vi "addEdge.vi"(0 "reference":refnum<class "CallNode.lvclass">, 1 "egde":refnum<class "AbstractEdge.lvclass">, 2 "p1":T1 {"y" format="%.2f"; "x" format="%.2f"}, 3 "p2":T1 {"y" format="%.2f"; "x" format="%.2f"}, 5 "error in (no error)":errorcluster) -> (14 "reference out":refnum<class "CallNode.lvclass">, 15 "edgeHasEndNode":bool, 19 "error out":errorcluster)   [LabVIEW 2020, in "CallNode.lvclass"]
uses:
  <resource>/Framework/Providers/Open_GDS/UML/CallNode_class/CallNode.lvclass
  C:/Program Files (x86)/National Instruments/LabVIEW 2020/resource/Framework/Providers/Open_GDS/UML/AbstractNode_class/AbstractNode.lvclass
  C:/Program Files (x86)/National Instruments/LabVIEW 2020/resource/Framework/Providers/Open_GDS/UML/RectangularNode_class/RectangularNode.lvclass
  <resource>/Framework/Providers/Open_GDS/UML/AbstractEdge_class/AbstractEdge.lvclass
  <resource>/Framework/Providers/Open_GDS/UML/General/Point/Point Point2D.ctl
  <resource>/Framework/Providers/Open_GDS/UML/ImplicitParameterNode_class/ImplicitParameterNode.lvclass
  <resource>/Framework/Providers/Open_GDS/UML/SegmentedLineEdge_class/SegmentedLineEdge.lvclass
  <resource>/Framework/Providers/Open_GDS/UML/RectangularNode_class/RectangularNode.lvclass
  <resource>/Framework/Providers/Open_GDS/UML/AbstractNode_class/AbstractNode.lvclass
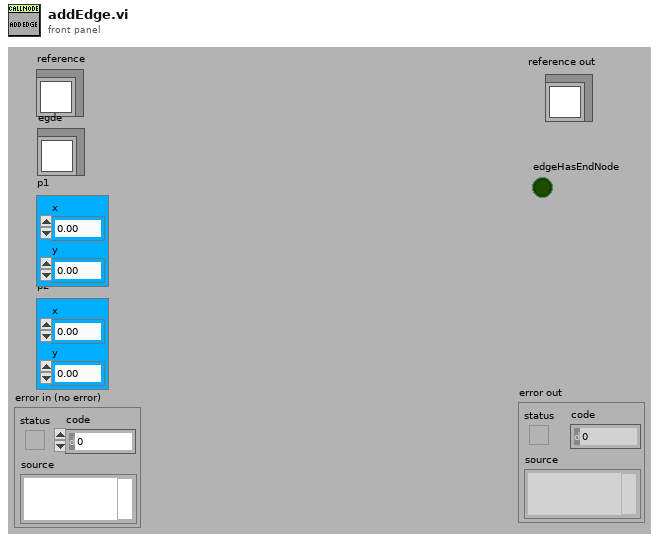
[diagram p1: front panel]
types:
  T1 = typedef "Point Point2D.ctl" = cluster{"x":dbl, "y":dbl}
  T2 = typedef "AbstractNode.lvclass/ObjectAttributes.ctl" = cluster{"parent":refnum<class "AbstractNode.lvclass">, "children":refnum<class "AbstractNode.lvclass">[], "Hidden":bool}
  T3 = typedef "Rectangle Rectangle2D.ctl" = cluster{"x":dbl, "y":dbl, "width":dbl, "height":dbl}
  T4 = typedef "CallNode.lvclass/ObjectAttributes.ctl" = cluster{"objectCallNodeRef":refnum<class "AbstractNode.lvclass">, "signaled":bool, "openBottom":bool, "DEFAULT_WIDTH":i32, "DEFAULT_HEIGHT":i32, "CALL_YGAP":i32}
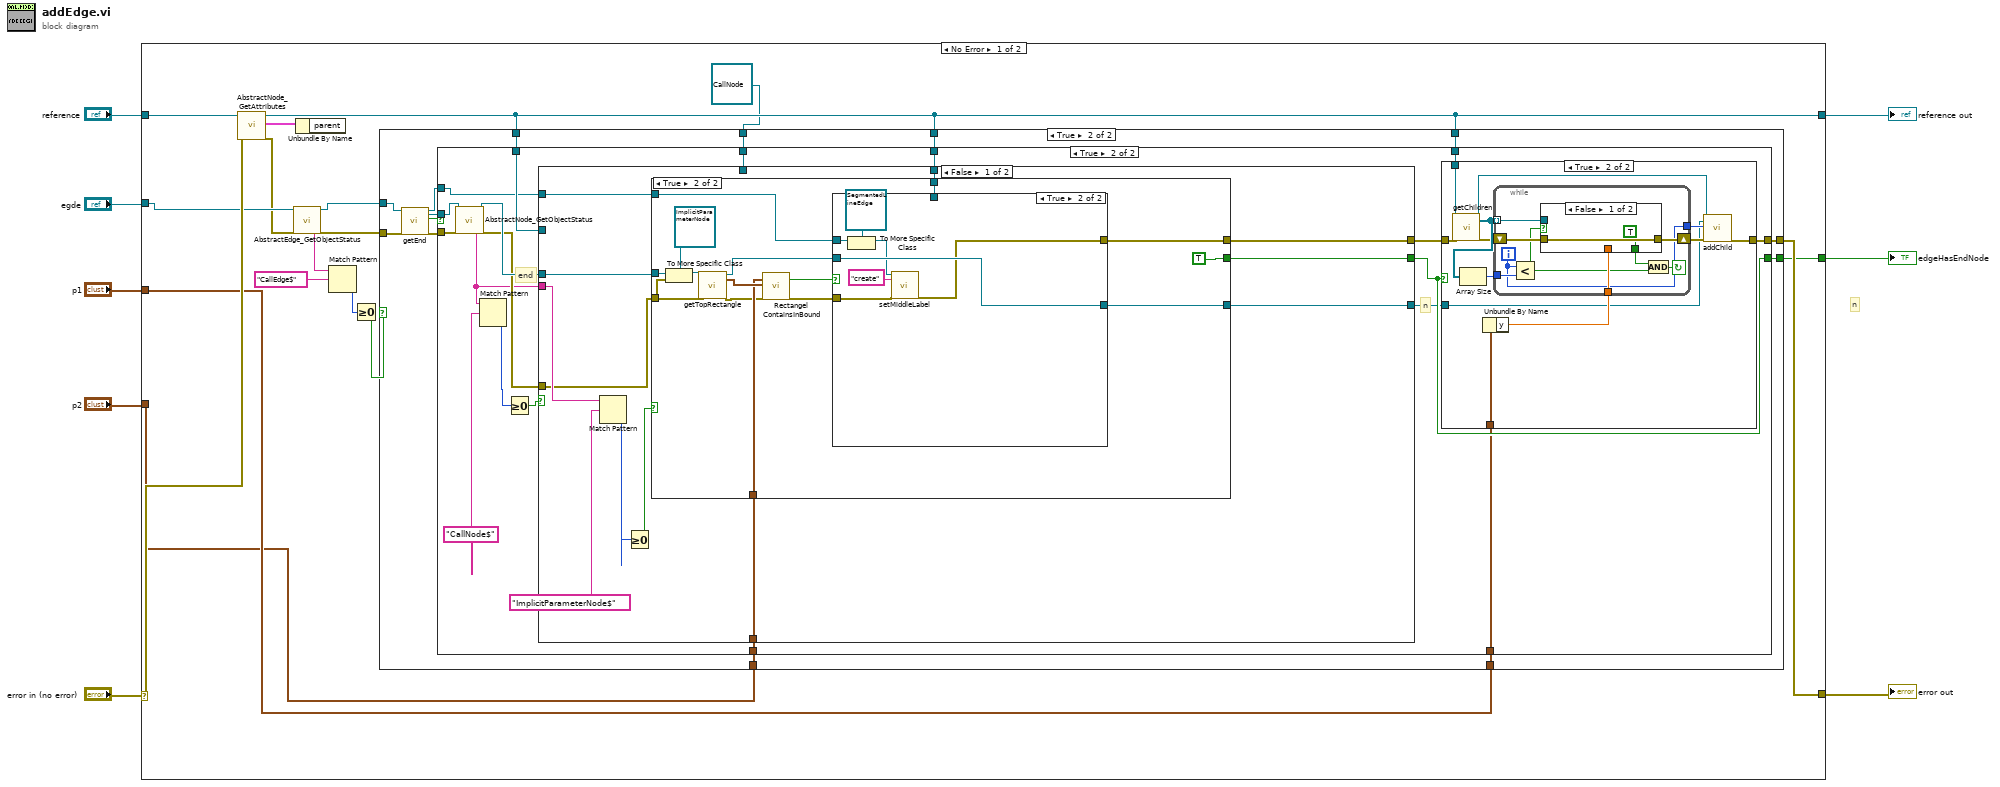
[diagram p0: block diagram]
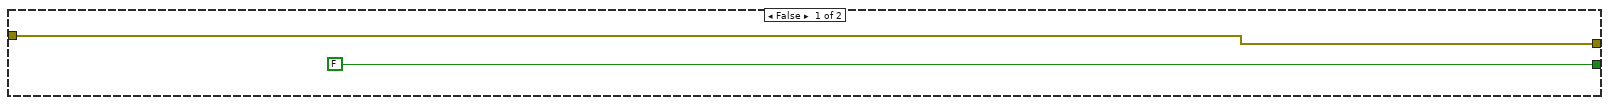
[diagram p2: hidden frame]
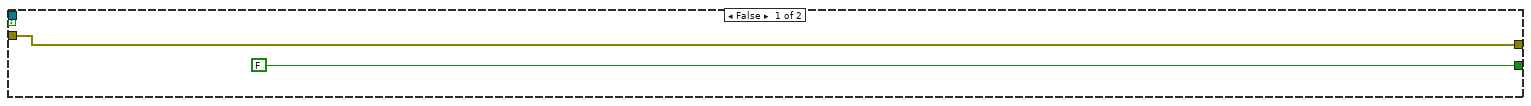
[diagram p3: hidden frame]
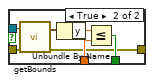
[diagram p5: hidden frame]
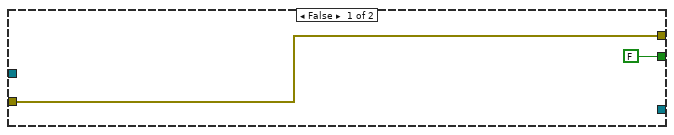
[diagram p6: hidden frame]
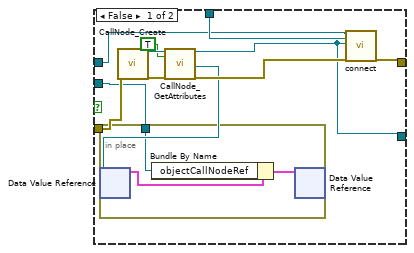
[diagram p7: hidden frame]
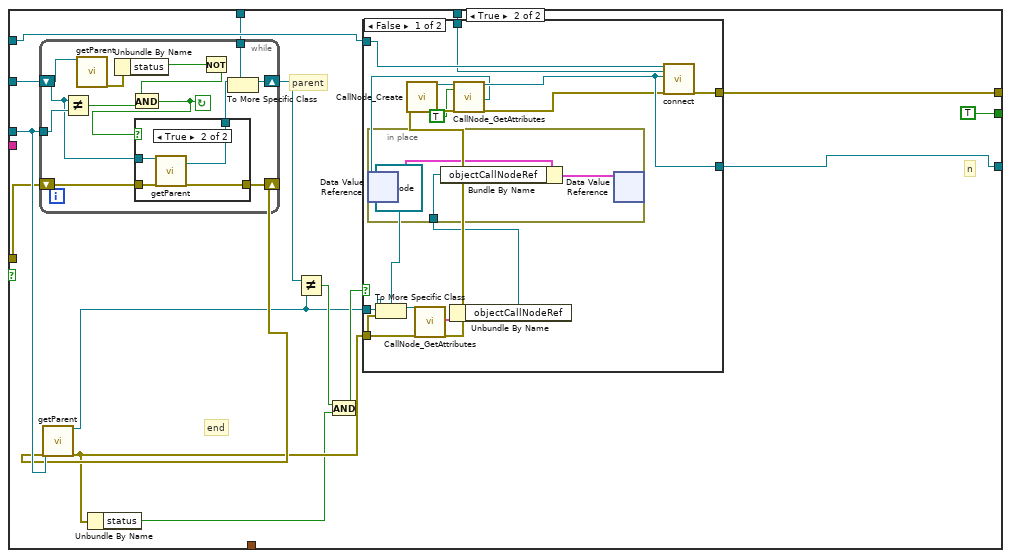
[diagram p8: hidden frame]
diagram:
  # "n"
  n1 = case shown="No Error" "error in (no error)" {
    selector: "error in (no error)" -> [w22 w199]
    tunnel: "reference" -> [w25 w200]
    tunnel: [w24 w199] -> w7
    tunnel: [w23 w200] -> w6
    tunnel: "egde" -> [w21 _]
    tunnel: [w20 _] -> w3
    tunnel: "p1" -> [w19 _]
    tunnel: "p2" -> [w18 _]
    frame No Error {
      n2 = call <resource>:"AbstractNode_GetAttributes.vi"("reference in"=w25, "error in (no error)"=w22) -> ("reference out"=w23:refnum<class "CallNode.lvclass">, "Data"=w10:T2, "error out"=w14:errorcluster)  [unwired: 14 in, 1 out]
      n3 = call <resource>:"AbstractEdge_GetObjectStatus.vi"("reference in"=w21, "error in (no error)"=w14) -> ("Class name"=w9:string, "reference out"=w13:refnum<class "AbstractEdge.lvclass">, "error out"=w12:errorcluster)  [unwired: 15 out]
      n4 = Unbundle By Name(w10) -> ()  [unwired: 1 out]
      n5 = Match Pattern(string=w9, regular expression="CallEdge$") -> (offset past match=w16:i32)  [unwired: 4 out]
      n6 = Greater Or Equal To 0?(x=w16) -> (x >= 0?=w15:bool)
      n7 = case shown="True" w15 {
        tunnel: [FALSE w41] -> w20
        tunnel: w13 -> [_ w40]
        tunnel: w12 -> [w26 w39]
        tunnel: w23 -> [_ w35]
        tunnel: w23 -> [_ w33]
        tunnel: w18 -> [_ w32]
        tunnel: w23 -> [_ w31]
        tunnel: w19 -> [_ w30]
        tunnel: [w26 w29] -> w24
        tunnel: refnum<class "CallNode.lvclass"> refnum ("reference out") -> [_ w28]
        frame False {
        }
        frame True {
          n8 = call-dynamic "getEnd.vi"("reference"=w40, "error in (no error)"=w39) -> ("reference out"=w34:refnum<class "AbstractEdge.lvclass">, "endNode"=w37:refnum<class "AbstractNode.lvclass">, "validNode"=w38:bool, "error out"=w36:errorcluster)  [unwired: 14 in]
          n9 = case shown="True" w38 {
            tunnel: [FALSE w50] -> w41
            tunnel: w37 -> [_ w62]
            tunnel: w36 -> [w42 w61]
            tunnel: w35 -> [_ w57]
            tunnel: w34 -> [_ w54]
            tunnel: w33 -> [_ w53]
            tunnel: w32 -> [_ w51]
            tunnel: w31 -> [_ w49]
            tunnel: w30 -> [_ w47]
            tunnel: [w42 w45] -> w29
            tunnel: w28 -> [_ w44]
            frame False {
            }
            frame True {
              # "n"
              # "end"
              n10 = call <resource>:"AbstractNode_GetObjectStatus.vi"("reference in"=w62, "error in (no error)"=w61) -> ("Class name"=w52:string, "reference out"=w56:refnum<class "AbstractNode.lvclass">, "error out"=w55:errorcluster)  [unwired: 15 out]
              n11 = Match Pattern(string=w52, regular expression="CallNode$") -> (offset past match=w60:i32)  [unwired: 4 out]
              n12 = Greater Or Equal To 0?(x=w60) -> (x >= 0?=w58:bool)
              n13 = case shown="False" w58 {
                tunnel: w57 -> [_ w159]
                tunnel: w56 -> [w100 w158]
                tunnel: w55 -> [w99 w155]
                tunnel: w54 -> [w96 w152]
                tunnel: w53 -> [w95 w151]
                tunnel: w52 -> [w103 _]
                tunnel: [w102 TRUE] -> w50
                tunnel: w51 -> [w98 _]
                tunnel: [w97 w149] -> w46
                tunnel: [w94 w147] -> w48
                tunnel: w44 -> [_ w146]
                frame False {
                  n14 = Match Pattern(string=w103, regular expression="ImplicitParameterNode$") -> (offset past match=w104:i32)  [unwired: 4 out]
                  n15 = Greater Or Equal To 0?(x=w104) -> (x >= 0?=w101:bool)
                  n16 = case shown="True" w101 {
                    tunnel: [FALSE TRUE] -> w102
                    tunnel: w100 -> [_ w110]
                    tunnel: w99 -> [w106 w111]
                    tunnel: w98 -> [_ w120]
                    tunnel: [_ w117] -> w97
                    tunnel: w96 -> [_ w115]
                    tunnel: w95 -> [_ w113]
                    tunnel: [w106 w112] -> w94
                    frame False {
                    }
                    frame True {
                      n17 = To More Specific Class(target class=refnum<class "ImplicitParameterNode.lvclass"> refnum ("reference"), reference=w110, error in=w111) -> (specific class reference=w108:refnum<class "ImplicitParameterNode.lvclass">)  [unwired: 1 out]
                      n18 = call-dynamic "getTopRectangle.vi"("reference"=w108, "error in (no error)"=w111) -> ("reference out"=w116:refnum<class "ImplicitParameterNode.lvclass">, "bounds"=w121:T3, "error out"=w119:errorcluster)  [unwired: 15 in]
                      n19 = call <resource>:"Rectangel ContainsInBound.vi"("point2D"=w120, "bounds"=w121, "error in (no error)"=w119) -> ("contains"=w118:bool, "error out"=w114:errorcluster)  [unwired: 1 in, 14 out]
                      n20 = case shown="True" w118 {
                        tunnel: [w127 w141] -> w117
                        tunnel: w116 -> [w123 w141]
                        tunnel: w115 -> [w128 w138]
                        tunnel: w114 -> [w131 w143]
                        tunnel: w113 -> [w129 _]
                        tunnel: [w126 w140] -> w112
                        frame False {
                          n21 = call <resource>:"CallNode_Create.vi"("error in (no error)"=w131) -> ("reference out"=w133:refnum<class "CallNode.lvclass">, "error out"=w132:errorcluster)  [unwired: 1 in, 16 out]
                          n22 = call <resource>:"CallNode_GetAttributes.vi"("reference in"=w133, "OnlyGetDvrReference(False)"=TRUE, "error in (no error)"=w132) -> ("reference out"=w127:refnum<class "CallNode.lvclass">, "DataRef"=w124:refnum<data-value>, "error out"=w130:errorcluster)  [unwired: 13 in, 1 out]
                          n23 = in-place {
                            in-place-border: w123 -> [w135]
                            n24 = in-place-dvr #1(w124) -> (w136:T4)  [unwired: 1 out]
                            n25 = Bundle By Name(cluster=w136, "objectCallNodeRef"=w135) -> (w134:T4)
                            n26 = in-place-dvr #1(w134) -> ()  [unwired: 2 out]
                          }
                          n27 = call-dynamic "connect.vi"("reference"=w128, "startNode"=w129, "endNode"=w127, "error in (no error)"=w130) -> ("error out"=w126:errorcluster)  [unwired: 14 in, 1 out]
                        }
                        frame True {
                          n28 = To More Specific Class(target class=refnum<class "SegmentedLineEdge.lvclass"> refnum ("reference"), reference=w138) -> (specific class reference=w137:refnum<class "SegmentedLineEdge.lvclass">)  [unwired: 1 in, 1 out]
                          n29 = call-dynamic "setMiddleLabel.vi"("reference"=w137, "middleLabel"="create", "error in (no error)"=w143) -> ("error out"=w140:errorcluster)  [unwired: 15 in, 1 out]
                        }
                      }
                    }
                  }
                }
                frame True {
                  # "parent"
                  # "end"
                  # "n"
                  n30 = while {
                    shift-right: [w185] -> w157
                    shift-left: w159 -> [w184]
                    tunnel: w158 -> [w192]
                    shift-right: [w188] -> w156
                    shift-left: w155 -> [w189]
                    tunnel: w146 -> [w186]
                    stop <- w190 continue-if-true
                    n31 = Not Equal?(x=w184, y=w192) -> (x != y?=w191:bool)
                    n32 = call-dynamic "getParent.vi"("reference"=w184) -> ("error out"=w183:errorcluster)  [unwired: 14 in, 4 out]
                    n33 = Unbundle By Name(w183) -> ("status"=w182:bool)
                    n34 = Not(x=w182) -> (.not. x?=w181:bool)
                    n35 = And(x=w181, y=w191) -> (x .and. y?=w190:bool)
                    n36 = case shown="True" w190 {
                      tunnel: w184 -> [w194 w198]
                      tunnel: [w194 w197] -> w187
                      tunnel: w189 -> [w193 w196]
                      tunnel: [w193 w195] -> w188
                      frame False {
                      }
                      frame True {
                        n37 = call-dynamic "getParent.vi"("reference"=w198, "error in (no error)"=w196) -> ("parentNode"=w197:refnum<class "AbstractNode.lvclass">, "error out"=w195:errorcluster)  [unwired: 13 in, 3 out]
                      }
                    }
                    n38 = To More Specific Class(target class=w186, reference=w187) -> (specific class reference=w185:refnum<class "CallNode.lvclass">)  [unwired: 1 in, 1 out]
                  }
                  n39 = call-dynamic "getParent.vi"("reference"=w158, "error in (no error)"=w156) -> ("reference out"=w150:refnum<class "AbstractNode.lvclass">, "error out"=w145:errorcluster)  [unwired: 13 in, 3 out]
                  n40 = Unbundle By Name(w145) -> ("status"=w144:bool)
                  n41 = Not Equal?(x=w157, y=w150) -> (x != y?=w154:bool)
                  n42 = And(x=w154, y=w144) -> (x .and. y?=w153:bool)
                  n43 = case shown="False" w153 {
                    tunnel: w150 -> [w166 w180]
                    tunnel: [w171 w180] -> w149
                    tunnel: w152 -> [w173 _]
                    tunnel: w151 -> [w172 _]
                    tunnel: w145 -> [w167 w179]
                    tunnel: [w168 w179] -> w147
                    frame False {
                      n44 = To More Specific Class(target class=refnum<class "CallNode.lvclass"> refnum ("reference out"), reference=w166, error in=w167) -> (specific class reference=w165:refnum<class "CallNode.lvclass">)  [unwired: 1 out]
                      n45 = call <resource>:"CallNode_GetAttributes.vi"("reference in"=w165, "error in (no error)"=w167) -> ("Data"=w162:T4, "error out"=w170:errorcluster)  [unwired: 1 in, 15 out]
                      n46 = call <resource>:"CallNode_Create.vi"("error in (no error)"=w170) -> ("reference out"=w175:refnum<class "CallNode.lvclass">, "error out"=w174:errorcluster)  [unwired: 1 in, 16 out]
                      n47 = Unbundle By Name(w162) -> ("objectCallNodeRef"=w160:refnum<class "AbstractNode.lvclass">)
                      n48 = call <resource>:"CallNode_GetAttributes.vi"("reference in"=w175, "OnlyGetDvrReference(False)"=TRUE, "error in (no error)"=w174) -> ("reference out"=w171:refnum<class "CallNode.lvclass">, "DataRef"=w161:refnum<data-value>, "error out"=w169:errorcluster)  [unwired: 13 in, 1 out]
                      n49 = in-place {
                        in-place-border: w160 -> [w177]
                        n50 = in-place-dvr #2(w161) -> (w178:T4)  [unwired: 1 out]
                        n51 = Bundle By Name(cluster=w178, "objectCallNodeRef"=w177) -> (w176:T4)
                        n52 = in-place-dvr #2(w176) -> ()  [unwired: 2 out]
                      }
                      n53 = call-dynamic "connect.vi"("reference"=w173, "startNode"=w172, "endNode"=w171, "error in (no error)"=w169) -> ("error out"=w168:errorcluster)  [unwired: 14 in, 1 out]
                    }
                    frame True {
                    }
                  }
                }
              }
              n54 = case shown="True" w50 {
                tunnel: w49 -> [_ w75]
                tunnel: w48 -> [w63 w74]
                tunnel: w47 -> [_ w70]
                tunnel: w46 -> [_ w65]
                tunnel: [w63 w64] -> w45
                frame False {
                }
                frame True {
                  n55 = call-dynamic "getChildren.vi"("reference"=w75, "error in (no error)"=w74) -> ("reference out"=w67:refnum<class "CallNode.lvclass">, "children"=w73:refnum<class "AbstractNode.lvclass">[], "error out"=w71:errorcluster)  [unwired: 14 in, 1 out]
                  n56 = Array Size(array=w73) -> (size(s)=w72:i32)
                  n57 = Unbundle By Name(w70) -> ("y"=w69:dbl)
                  n58 = while {
                    shift-right: [w78] -> w68
                    shift-left: w71 -> [w83]
                    tunnel: w73 -> [w82] mode=indexing
                    tunnel: w72 -> [w84]
                    tunnel: w69 -> [w81]
                    tunnel: [w77] -> w66
                    i -> [w77]
                    stop <- w79 continue-if-true
                    n59 = Less?(x=w77, y=w84) -> (x < y?=w76:bool)
                    n60 = case shown="False" w76 {
                      tunnel: w83 -> [w86 w93]
                      tunnel: w82 -> [_ w92]
                      tunnel: w81 -> [_ w89]
                      tunnel: [TRUE w88] -> w80
                      tunnel: [w86 w87] -> w78
                      frame False {
                      }
                      frame True {
                        n61 = call-dynamic "getBounds.vi"("reference"=w92, "error in (no error)"=w93) -> ("bounds"=w91:T3, "error out"=w87:errorcluster)  [unwired: 15 in, 1 out]
                        n62 = Unbundle By Name(w91) -> ("y"=w90:dbl)
                        n63 = Less Or Equal?(x=w90, y=w89) -> (x <= y?=w88:bool)
                      }
                    }
                    n64 = And(x=w80, y=w76) -> (x .and. y?=w79:bool)
                  }
                  n65 = call-dynamic "addChild.vi"("reference"=w67, "node"=w65, "index(last)"=w66, "error in (no error)"=w68) -> ("error out"=w64:errorcluster)  [unwired: 14 in, 1 out]
                }
              }
            }
          }
        }
      }
    }
    frame Error {
    }
  }
  "reference out" <- w6
  "error out" <- w7
  "edgeHasEndNode" <- w3
